vi "FX_Sum.vi"(11 "Body":string) -> (3 "SS":string)   [LabVIEW 2018]
doc: "Use this template to build a VI to use as a subVI."
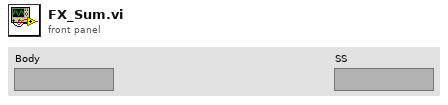
[diagram p1: front panel]
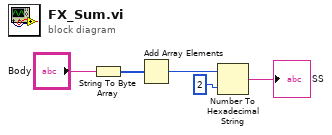
[diagram p0: block diagram]
diagram:
  n1 = String To Byte Array(string="Body") -> (unsigned byte array=w4:u8[])
  n2 = Add Array Elements(numeric array=w4) -> (sum=w3:u8)
  n3 = Number To Hexadecimal String(1:i16 2 ("width (-)"), 2:w3) -> (0:→"SS":string)
